vi "On Success.vi"(8 "error in (no error)":errorcluster, 9 "Session In":refnum<class "Session.lvclass">, 10 "User":refnum<class "User.lvclass">, 11 "FormAuthentication in":refnum<class "FormAuthentication.lvclass">) -> (0 "error out":errorcluster, 1 "Session":refnum<class "Session.lvclass">, 2 "Response":refnum<class "Response.lvclass">, 3 "FormAuthentication out":refnum<class "FormAuthentication.lvclass">)   [LabVIEW 2020, in "HTTP Server.lvlib" / "FormAuthentication.lvclass"]
uses:
  FormAuthentication.lvclass
  lv-http-util/HTTP Utils/Response/Response.lvclass
  Session/Session.lvclass
  User/User.lvclass
  Authentication Provider/Authentication Provider.lvclass
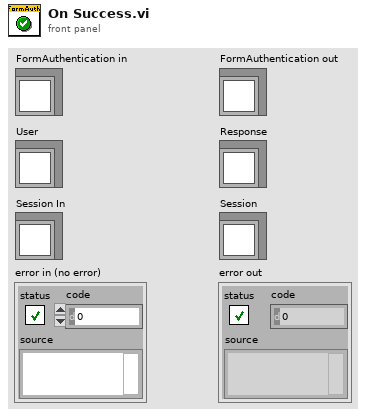
[diagram p1: front panel]
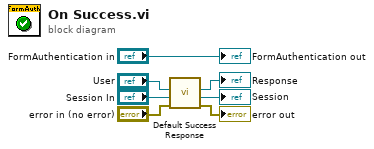
[diagram p0: block diagram]
diagram:
  n1 = call "Default Success Response.vi"("error in (no error)"="error in (no error)", "Session In"="Session In", "User"="User") -> ("error out"=→"error out":errorcluster, "Session"=→"Session":refnum<class "Session.lvclass">, "Response"=→"Response":refnum<class "Response.lvclass">)  [unwired: 6 in]
  "FormAuthentication out" <- "FormAuthentication in"
